vi "Assert Less Or Equal_Variant.vi"(4 "Execution time (s)":dbl=-1.0, 5 "Assert Only? (F)":bool, 6 "error code (1)":i32=1, 7 "Label":string, 8 "error in (no error)":errorcluster, 9 "Register with caller test (F)":bool, 10 "Y":variant, 11 "X":variant) -> (0 "error out":errorcluster, 2 "Properties.Assert":refnum<class "Properties.Assert.lvclass">)   [LabVIEW 2020, in "Caraya.lvlib" / "Assert.lvclass"]
doc: "Generates an error if the input condition is not met.\n\n--\nCopyright © 2015 JKI All rights reserved.\n\nAuthor: Tomi Maila <tomi.maila@jki.net>\n\nThis library is provided \"AS IS\" ,WITHOUT WARRANTIES OR\nCONDITIONS OF ANY KIND, either express or implied.\n\nJKI -- jki.net"
uses:
  Assert.lvclass
  Assert.lvclass/Assert.ctl
  <userlib>/_OpenG.lib/string/string.llb/openg_string.lvlib
  Properties/Properties.lvclass
  Properties.Assert/Properties.Assert.lvclass
  C:/Projects/caraya/src/classes/Properties/Properties.lvclass
  C:/Projects/caraya/src/classes/Properties.Assert/Properties.Assert.lvclass
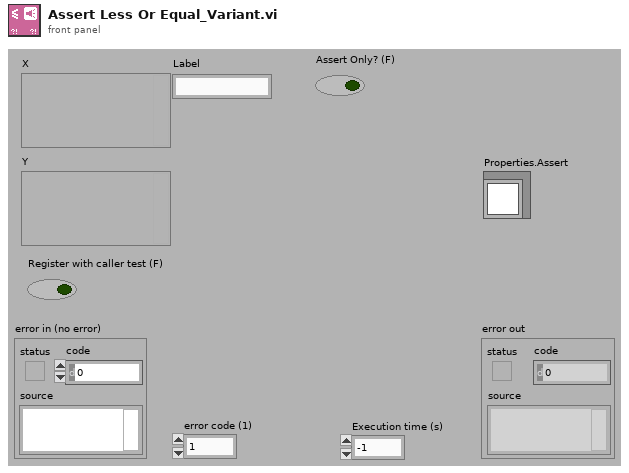
[diagram p1: front panel]
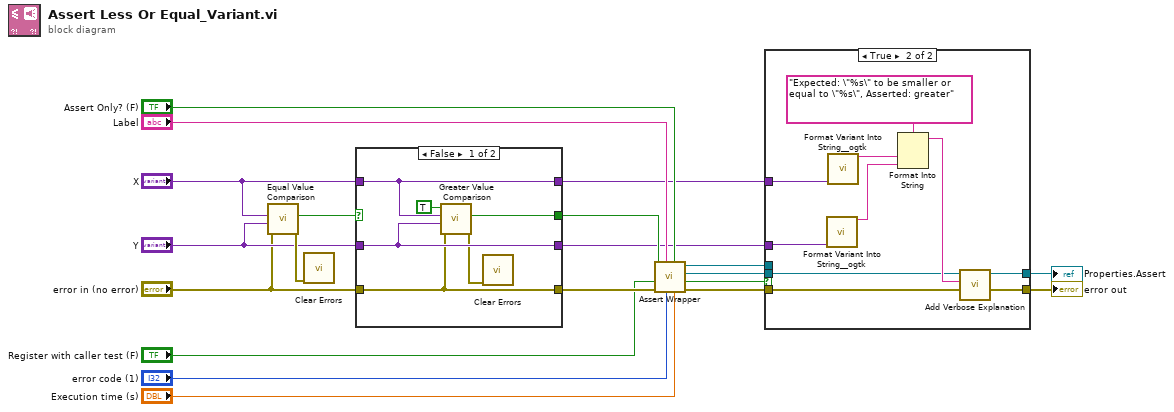
[diagram p0: block diagram]
diagram:
  n1 = call "Equal Value Comparison.vi"("error in (no error)"="error in (no error)", "Actual"="Y", "Expected"="X") -> ("error out"=w12:errorcluster, "Equal Values?"=w13:bool)  [unwired: 6 in, 1 out]
  n2 = call <vilib>:"Clear Errors.vi"("error in (no error)"=w12) -> ()  [unwired: 5 in, 2 out]
  n3 = case shown="False" w13 {
    selector: w13 -> [_ w29]
    tunnel: "X" -> [w26 w30]
    tunnel: [w26 w30] -> w9
    tunnel: [w24 w29] -> w10
    tunnel: "Y" -> [w25 w28]
    tunnel: [w25 w28] -> w6
    tunnel: "error in (no error)" -> [w23 w27]
    tunnel: [w23 w27] -> w11
    frame False {
      n4 = call "Greater Value Comparison.vi"("error in (no error)"=w23, "Y"=w25, "X"=w26, "Less Than? (F)"=TRUE) -> ("error out"=w22:errorcluster, "Asserted?"=w24:bool)  [unwired: 5 in, 1 out]
      n5 = call <vilib>:"Clear Errors.vi"("error in (no error)"=w22) -> ()  [unwired: 5 in, 2 out]
    }
    frame True {
    }
  }
  n6 = call "Assert Wrapper.vi"("Execution time (s)"="Execution time (s)", "Assert Only? (F)"="Assert Only? (F)", "error code (1)"="error code (1)", "Label"="Label", "error in (no error)"=w11, "Register with caller test (F)"="Register with caller test (F)", "Assert?"=w10) -> ("error out"=w16:errorcluster, "Verbose"=w14:bool, "Properties.Assert"=w2:refnum<class "Properties.Assert.lvclass">, "Assert out"=w3:refnum<class "Assert.lvclass">)  [unwired: 1 in]
  n7 = case shown="True" w14 {
    tunnel: [w32 w36] -> w15
    tunnel: w3 -> [_ _]
    tunnel: w16 -> [w32 w37]
    tunnel: w9 -> [_ w42]
    tunnel: w6 -> [_ w41]
    tunnel: w2 -> [w31 w34]
    tunnel: [w31 w33] -> w1
    frame False {
    }
    frame True {
      n8 = call <userlib>:"Format Variant Into String__ogtk.vi"("Variant"=w41) -> ("Output String"=w38:string)  [unwired: 13 in, 1 out]
      n9 = call <userlib>:"Format Variant Into String__ogtk.vi"("Variant"=w42) -> ("Output String"=w39:string)  [unwired: 13 in, 1 out]
      n10 = Format Into String(format string="Expected: \"%s\" to be smaller or equal to \"%s\", Asserted: greater" ("t"), w39, w38) -> (resulting string=w35:string)  [unwired: 2 in, 1 out]
      n11 = call "Add Verbose Explanation.vi"("error in (no error)"=w37, "Verbose Explanation"=w35, "Properties"=w34) -> ("error out"=w36:errorcluster, "Properties"=w33:refnum<class "Properties.Assert.lvclass">)  [unwired: 7 in]
    }
  }
  "error out" <- w15
  "Properties.Assert" <- w1
